vi "Get Reserved Names.vi"() -> (2 "reserved names":string[](array[string])=["InstrumentStudio Plugin SDK"])   [LabVIEW 2021, in "InstrumentStudio Plug-In Editor.lvlib"]
uses:
  InstrumentStudio Plug-In Editor.lvlib
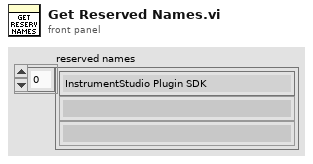
[diagram p1: front panel]
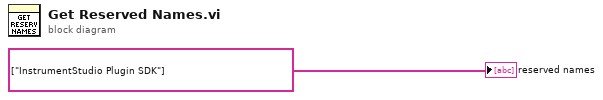
[diagram p0: block diagram]
diagram:
  "reserved names" <- string[] ["InstrumentStudio Plugin SDK"] ("Libraries from MeasurementLink Runtime")
